vi "Set MCP Request Context.vi"(8 "error in":errorcluster, 9 "stream":string, 10 "request":string, 11 "MCP Request Metadata":T1) -> (0 "error out":errorcluster, 1 "input requests queue":refnum<queue>, 2 "context queue":refnum<queue>, 3 "request out":string)   [LabVIEW 2020, in "MCP Server.lvlib"]
doc: "Publishes the context of the request about to be handled, so that Ask User.vi can read it while a tool runs: {\"era\",\"elicitation\",\"inputResponses\",\"id\",\"progressToken\",\"stream\"} becomes the only element of the named queue \"MCP Request Context\". The queue has size 1, which also serialises request handling: the enqueue waits while another request still holds the context. Questions left over in the named queue \"MCP Input Requests\" are discarded.\n\nera is \"modern\" or \"legacy\"; elicitation is true only for a modern request whose clientCapabilities carry elicitation. id is the id of MCP Request Metadata (the JSON text of the request id, null when missing). progressToken is params._meta.progressToken of the request as JSON text, null when missing. stream is the stream input, null when it is empty. Report Progress.vi and Cancel Requested.vi read id, progressToken and stream from the context.\n\nBoth queue references stay open and go to Collect MCP Input Requests.vi, which takes the context out again and releases them. request out is request, passed on only once the context is in place, so that the request handler that consumes it runs after this.\n\nQueue errors do not stop the request and are discarded, as before the split; so is the error of looking up progressToken. error in is passed through unchanged."
uses:
  MCP Server.lvlib
  MCP Request Metadata.ctl
  <vilib>/JDP Science/JSONtext/Next JSON Value.vi
  <vilib>/JDP Science/JSONtext/String Subset.vi
  <vilib>/JDP Science/JSONtext/Parsing/Advance past next JSON Value (inlined COPY).vi
  <vilib>/JDP Science/JSONtext/Parsing/Advance past whitespace.vi
  <vilib>/JDP Science/JSONtext/Parsing/Advance past String.vi
  <vilib>/JDP Science/JSONtext/Parsing/Advance past Number.vi
  <vilib>/JDP Science/JSONtext/Parsing/Advance past Line Ending.vi
  <vilib>/JDP Science/JSONtext/Parsing/Parse Full Path or Item Name.vi
  <vilib>/JDP Science/JSONtext/Parsing/Advance past Array.vi
  <vilib>/JDP Science/JSONtext/Parsing/Advance past Object.vi
  <vilib>/JDP Science/JSONtext/support/Error Cluster From Code.vi
  <vilib>/JDP Science/JSONtext/Offset/Find Item Locations by Path.vi
  <vilib>/JDP Science/JSONtext/JSONtext.lvlib
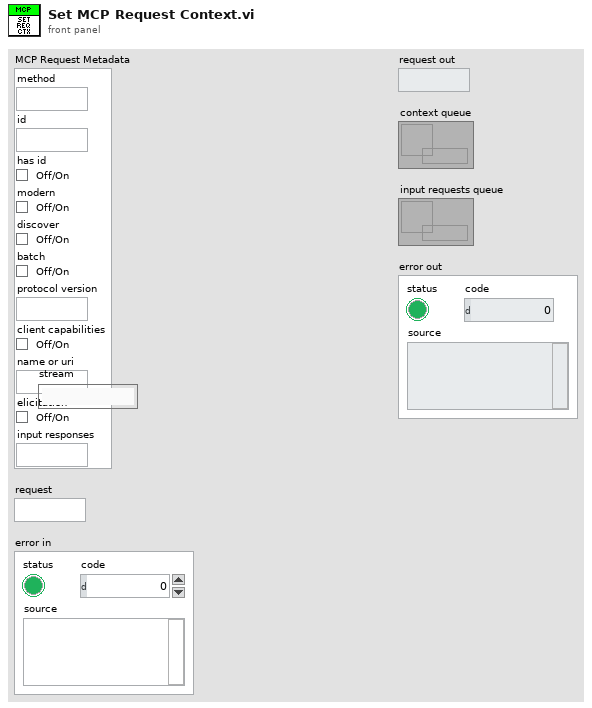
[diagram p1: front panel]
types:
  T1 = typedef "MCP Server.lvlib/MCP Request Metadata.ctl" = cluster{"method":string, "id":string, "has id":bool, "modern":bool, "discover":bool, "batch":bool, "protocol version":string, "client capabilities":bool, "name or uri":string, "elicitation":bool, "input responses":string}
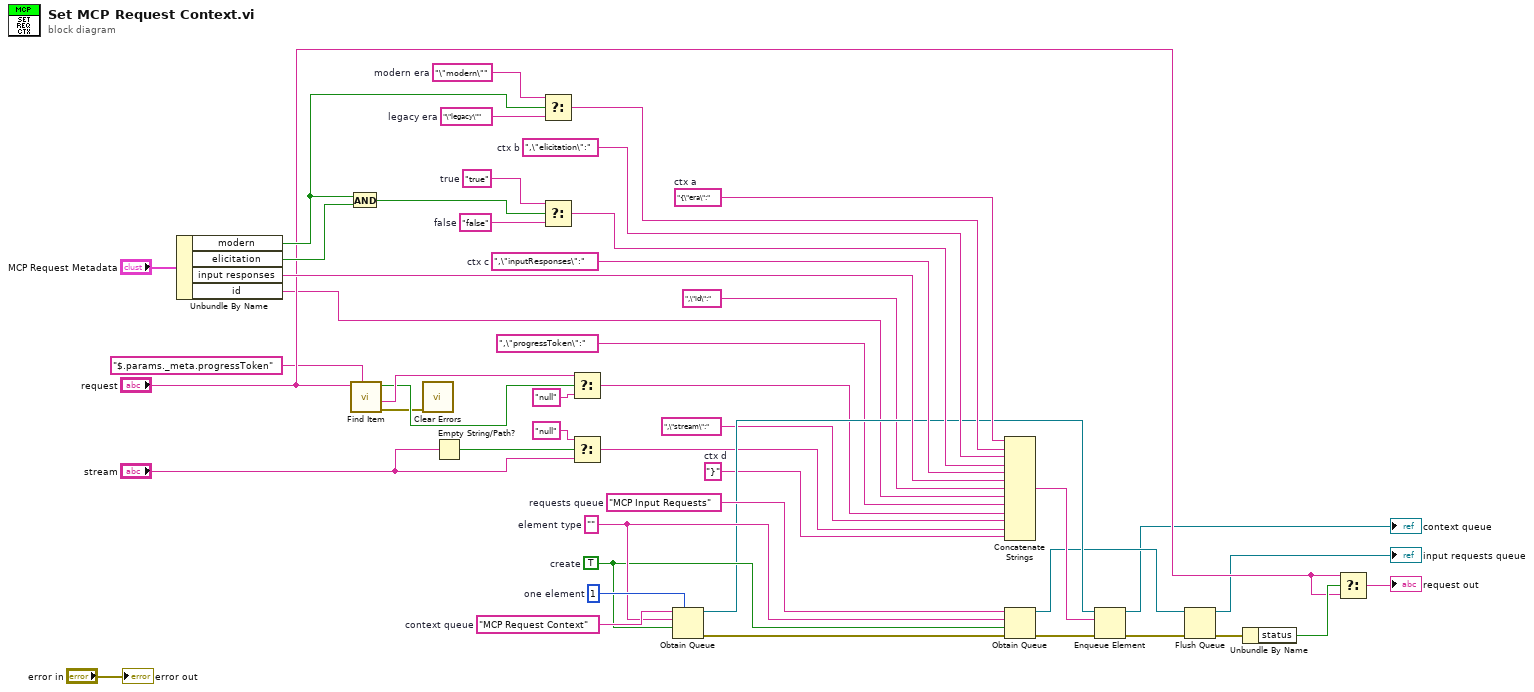
[diagram p0: block diagram]
diagram:
  w44 = "MCP Input Requests"  # requests queue
  w46 = "MCP Request Context"  # context queue
  w45 = 1  # one element
  w42 = TRUE  # create
  w43 = ""  # element type
  w1 = "}"  # ctx d
  w29 = ",\"inputResponses\":"  # ctx c
  w31 = ",\"elicitation\":"  # ctx b
  w33 = "{\"era\":"  # ctx a
  w34 = "false"  # false
  w36 = "true"  # true
  w39 = "\"legacy\""  # legacy era
  w40 = "\"modern\""  # modern era
  n1 = Unbundle By Name("MCP Request Metadata") -> ("modern"=w38:bool, "elicitation"=w37:bool, "input responses"=w28:string, "id"=w6:string)
  n2 = And(x=w38, y=w37) -> (x .and. y?=w35:bool)
  n3 = call <vilib>:"Find Item.vi"("$Path or Item Name"="$.params._meta.progressToken", "JSON"="request") -> ("error out"=w11:errorcluster, "<JSON>"=w14:string, "Found"=w13:bool)  [unwired: 6 in, 1 out]
  n4 = call <vilib>:"Clear Errors.vi"("error in (no error)"=w11) -> ()  [unwired: 5 in, 2 out]
  n5 = Empty String/Path?(string/path="stream") -> (empty?=w9:bool)
  n6 = Select(t=w40, s=w38, f=w39) -> (s? t:f=w32:string)
  n7 = Select(t=w36, s=w35, f=w34) -> (s? t:f=w30:string)
  n8 = Select(t=w14, s=w13, f="null") -> (s? t:f=w4:string)
  n9 = Select(t="null", s=w9, f="stream") -> (s? t:f=w2:string)
  n10 = Obtain Queue(max queue size (-1, unlimited)=w45, name (unnamed)=w46, element data type=w43, create if not found? (T)=w42) -> (queue out=w27:refnum<queue>, error out=w41:errorcluster)  [unwired: 1 in, 1 out]
  n11 = Concatenate Strings(w33, w32, w31, w30, w29, w28, ",\"id\":" ("string"), w6, ",\"progressToken\":" ("string"), w4, ",\"stream\":" ("string"), w2, w1) -> (w26:string)
  n12 = Obtain Queue(name (unnamed)=w44, element data type=w43, create if not found? (T)=w42, error in (no error)=w41) -> (queue out=w24:refnum<queue>, error out=w25:errorcluster)  [unwired: 1 in, 1 out]
  n13 = Enqueue Element(queue=w27, element=w26, error in (no error)=w25) -> (queue out=→"context queue":refnum<queue>, error out=w23:errorcluster)  [unwired: 1 in, 1 out]
  n14 = Flush Queue(queue=w24, error in (no error)=w23) -> (queue out=→"input requests queue":refnum<queue>, error out=w22:errorcluster)  [unwired: 1 out]
  n15 = Unbundle By Name(w22) -> ("status"=w21:bool)
  n16 = Select(t="request", s=w21, f="request") -> (s? t:f=→"request out":string)
  "error out" <- "error in"
